vi "Beer_Pong_selecteur.vi"(0 "Espace dispo":dbl[][](array[numeric]), 1 "Timeout Count":u32, 5 "Zone 3":dbl[][](array[numeric]), 7 "Zone 2":dbl[][](array[numeric])=[[0.0, 1.0, 2.0, 3.0, 4.0, 32.0, 33.0, 36.0], [15.0, 30.0, 18.0, 24.0, 26.0, 13.0, 16.0, 19.0], [1.0, 0.0, 0.0, 0.0, 0.0, 0.0, 0.0, 0.0]], 11 "error in (no error)":errorcluster, 12 "Tick Count(mSec)":u32, 13 "New Angle":dbl) -> (4 "Selection de état":T2, 6 "Timeout Count":u32, 8 "Tick Count(mSec)":u32, 10 "New Angle":dbl, 14 "Timeout":bool=TRUE, 15 "error out":errorcluster)   [LabVIEW 2017]
uses:
  enum_etats_lidar.ctl
  enum_etats_beer_pong.ctl
panel:
  in  "Enum etat beer pong":T1
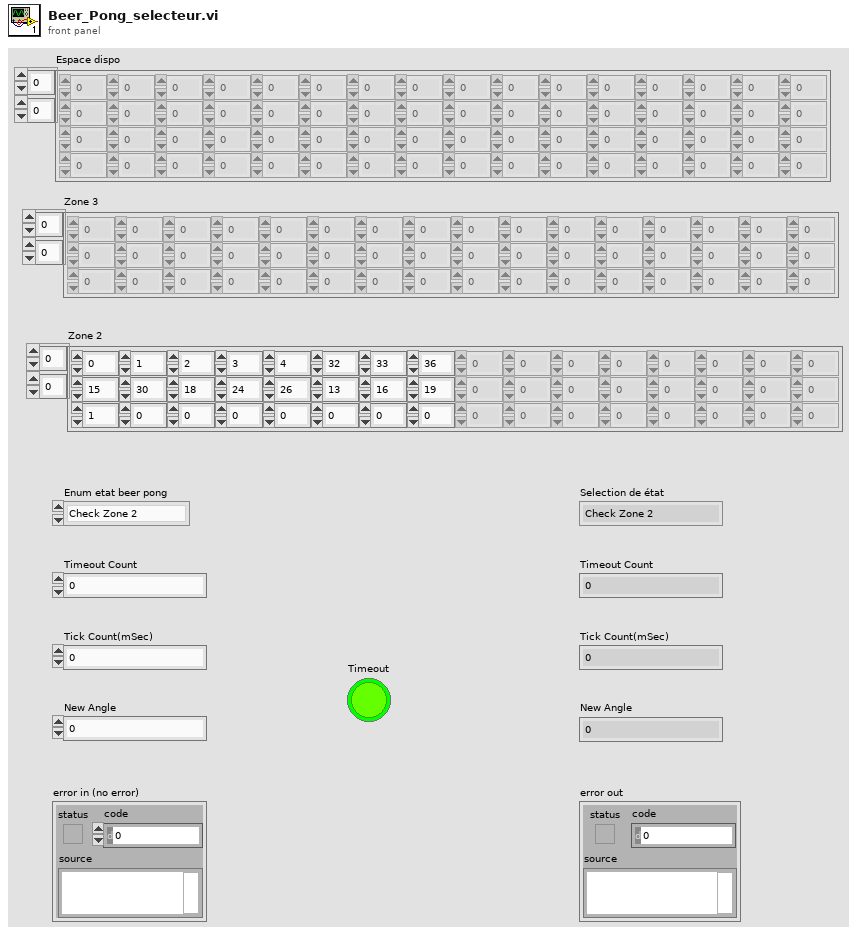
[diagram p1: front panel]
types:
  T1 = typedef "enum_etats_beer_pong.ctl" = enum16{"Check Zone 2", "Obstacle Zone 2", "Check Zone 3", "Obstacle Zone 3", "Avance", "Obstacle Timer", "Rescan 10s", "Check Zone 3 Bis", "Rotation new direction", "Rotation 180", "Timeout ?", "Arret complet", "Rotation new dir timer", "Rotation 180 timer"}
  T2 = typedef "enum_etats_lidar.ctl" = enum16{"Check Zone 2", "Obstacle Zone 2", "Check Zone 3", "Obstacle Zone 3", "Avance", "Obstacle Timer", "Rescan 10s", "Check Zone 3 Bis", "Rotation new direction", "Rotation 180", "Timeout ?", "Arret complet", "Rotation new dir timer", "Rotation 180 timer"}
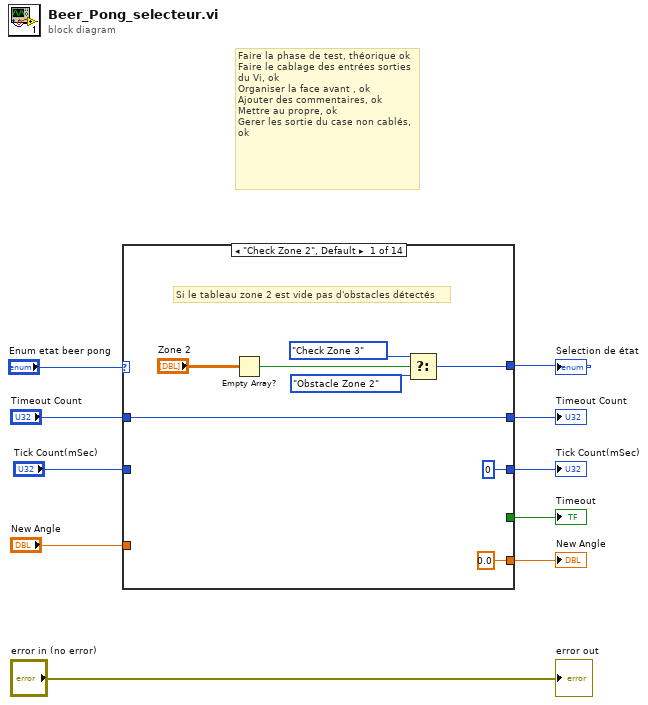
[diagram p0: block diagram]
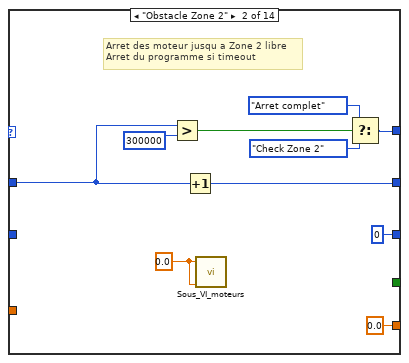
[diagram p2: hidden frame]
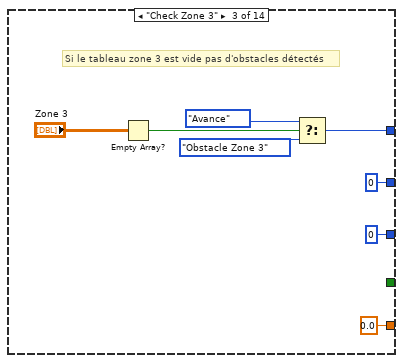
[diagram p3: hidden frame]
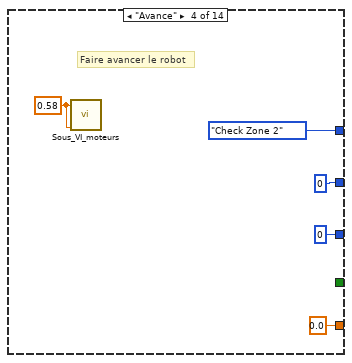
[diagram p4: hidden frame]
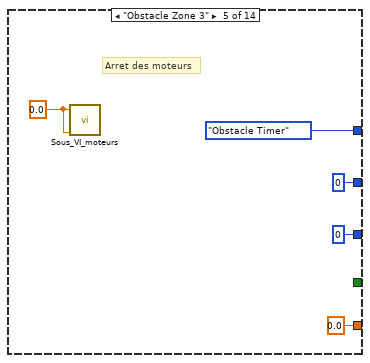
[diagram p5: hidden frame]
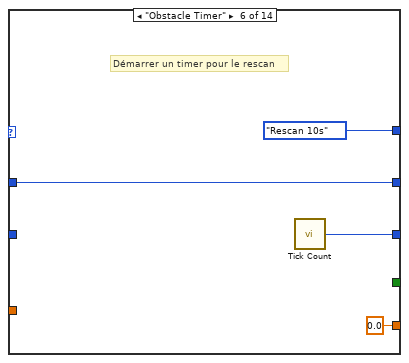
[diagram p6: hidden frame]
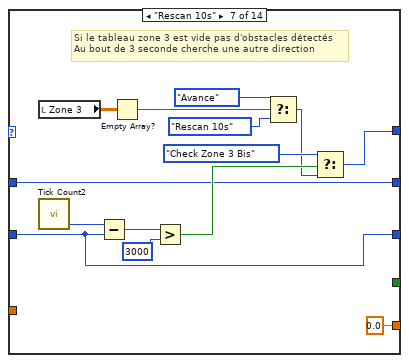
[diagram p7: hidden frame]
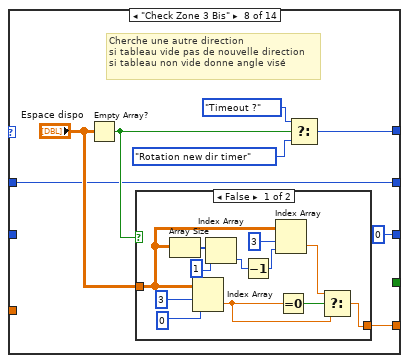
[diagram p8: hidden frame]
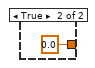
[diagram p9: hidden frame]
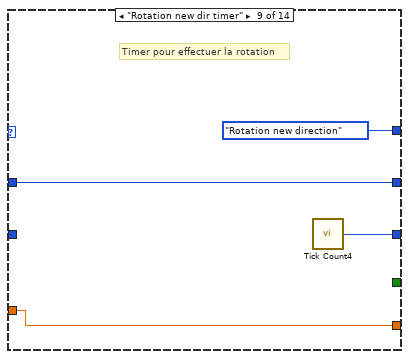
[diagram p10: hidden frame]
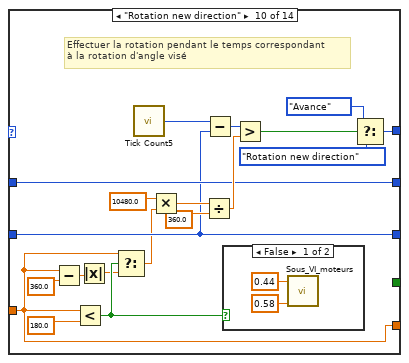
[diagram p11: hidden frame]
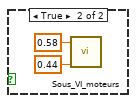
[diagram p12: hidden frame]
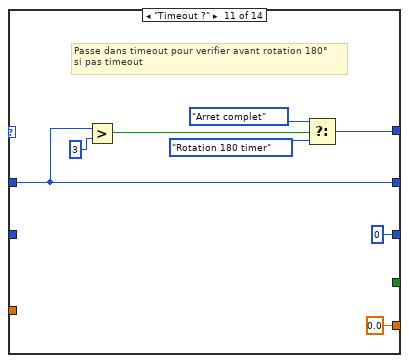
[diagram p13: hidden frame]
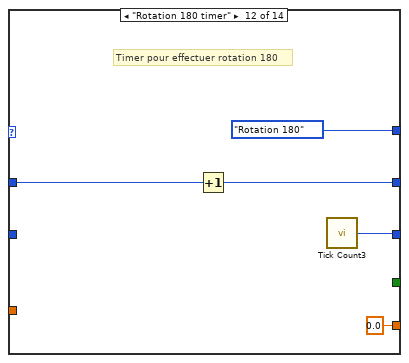
[diagram p14: hidden frame]
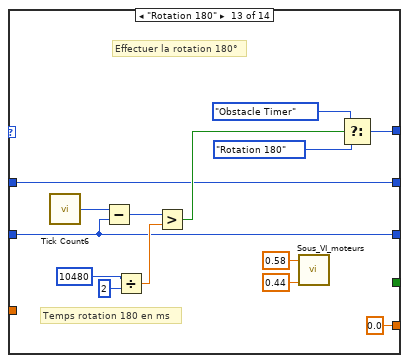
[diagram p15: hidden frame]
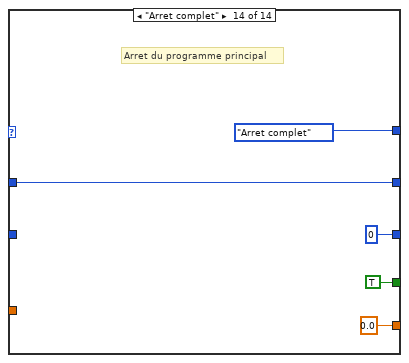
[diagram p16: hidden frame]
diagram:
  # "Faire la phase de test, théorique ok\nFaire le cablage des entrées sorties\ndu Vi, ok\nOrganiser la face avant , ok\nAjouter des commentaires, ok\nMettre au propre, ok\nGerer les sortie du case non cablés, ok"
  n1 = case shown="\"Check Zone 2\", Default" "Enum etat beer pong" {
    tunnel: [w14 w22 w32 enum_etats_lidar."Check Zone 2" ("Enum") enum_etats_lidar."Obstacle Timer" ("Enum") enum_etats_lidar."Rescan 10s" ("Enum") w51 w70 enum_etats_lidar."Rotation new direction" ("Enum") w106 w120 enum_etats_lidar."Rotation 180" ("Enum") w132 enum_etats_lidar."Arret complet" ("Enum")] -> w9
    tunnel: [u32 0 ("Tick Count(mSec)") u32 0 ("Tick Count(mSec)") u32 0 ("Tick Count(mSec)") u32 0 ("Tick Count(mSec)") u32 0 ("Tick Count(mSec)") w50 w53 u32 0 ("Tick Count(mSec)") w88 w98 u32 0 ("Tick Count(mSec) 2") w124 w128 u32 0 ("Tick Count(mSec) 2")] -> w8
    tunnel: "Tick Count(mSec)" -> [_ _ _ _ _ _ w53 _ _ w98 _ _ w128 _]
    tunnel: [_ _ _ _ _ _ _ _ _ _ _ _ _ TRUE] -> w6
    tunnel: "Timeout Count" -> [w11 w23 _ _ _ w48 w54 w66 w87 w99 w115 w121 w126 w142]
    tunnel: [w11 w24 0 0 ("Timeout Count") 0 w48 w54 w66 w87 w99 w115 w122 w126 w142] -> w4
    tunnel: [0.0 ("New Angle") 0.0 ("New Angle") 0.0 ("New Angle") 0.0 ("New Angle") 0.0 ("New Angle") 0.0 ("New Angle") 0.0 ("New Angle") w68 w86 w91 0.0 ("New Angle") 0.0 ("New Angle") 0.0 ("New Angle") 0.0 ("New Angle")] -> w3
    tunnel: "New Angle" -> [_ _ _ _ _ _ _ _ w86 w91 _ _ _ _]
    frame "Check Zone 2", Default {
      # "Si le tableau zone 2 est vide pas d'obstacles détectés"
      n2 = Empty Array?(array="Zone 2") -> (empty?=w17:bool)
      n3 = Select(t=enum_etats_lidar."Check Zone 3" ("Enum"), s=w17, f=enum_etats_lidar."Obstacle Zone 2" ("Enum")) -> (s? t:f=w14:T2)
    }
    frame "Obstacle Zone 2" {
      w28 = 0.0 ("Moteur Gauche")
      # "Arret des moteur jusqu a Zone 2 libre\nArret du programme si timeout"
      n4 = Greater?(x=w23, y=u32 300000) -> (0:w19:bool)
      n5 = Increment(x=w23) -> (x+1=w24:u32)
      n6 = call "Sous_VI_moteurs.vi"("Moteur Droit"=w28, "Moteur Gauche"=w28) -> ()  [unwired: 10 in]
      n7 = Select(t=enum_etats_lidar."Arret complet" ("Enum"), s=w19, f=enum_etats_lidar."Check Zone 2" ("Enum")) -> (s? t:f=w22:T2)
    }
    frame "Check Zone 3" {
      # "Si le tableau zone 3 est vide pas d'obstacles détectés"
      n8 = Empty Array?(array="Zone 3") -> (empty?=w36:bool)
      n9 = Select(t=enum_etats_lidar."Avance" ("Enum"), s=w36, f=enum_etats_lidar."Obstacle Zone 3" ("Enum")) -> (s? t:f=w32:T2)
    }
    frame "Avance" {
      w40 = 0.58 ("Moteur Gauche")
      # "Faire avancer le robot"
      n10 = call "Sous_VI_moteurs.vi"("Moteur Droit"=w40, "Moteur Gauche"=w40) -> ()  [unwired: 10 in]
    }
    frame "Obstacle Zone 3" {
      w46 = 0.0 ("Moteur Gauche")
      # "Arret des moteurs"
      n11 = call "Sous_VI_moteurs.vi"("Moteur Droit"=w46, "Moteur Gauche"=w46) -> ()  [unwired: 10 in]
    }
    frame "Obstacle Timer" {
      # "Démarrer un timer pour le rescan"
      n12 = call "Tick Count"() -> ("Tick Count(mSec)"=w50:u32)
    }
    frame "Rescan 10s" {
      # "Si le tableau zone 3 est vide pas d'obstacles détectés\nAu bout de 3 seconde cherche une autre direction"
      n13 = local read "Zone 3"() -> (w61:dbl[][])
      n14 = call "Tick Count2"() -> ("Tick Count(mSec)"=w60:u32)
      n15 = Subtract(x=w60, y=w53) -> (x-y=w59:u32)
      n16 = Empty Array?(array=w61) -> (empty?=w64:bool)
      n17 = Greater?(x=w59, y=u32 3000) -> (0:w57:bool)
      n18 = Select(t=enum_etats_lidar."Avance" ("Enum"), s=w64, f=enum_etats_lidar."Rescan 10s" ("Enum")) -> (s? t:f=w55:T2)
      n19 = Select(t=enum_etats_lidar."Check Zone 3 Bis" ("Enum"), s=w57, f=w55) -> (s? t:f=w51:T2)
    }
    frame "Check Zone 3 Bis" {
      # "Cherche une autre direction\nsi tableau vide pas de nouvelle direction\nsi tableau non vide donne angle visé"
      n20 = Empty Array?(array="Espace dispo") -> (empty?=w69:bool)
      n21 = case shown="False" w69 {
        tunnel: [w78 0.0 ("Numeric")] -> w68
        tunnel: "Espace dispo" -> [w77 _]
        frame False {
          n22 = Array Size(array=w77) -> (size(s)=w76:i32[])
          n23 = Index Array(array=w77, index (row)=3, index (col)=0 ("disabled index (col)")) -> (element=w81:dbl)
          n24 = Index Array(array=w76, index=1) -> (element=w73:i32)
          n25 = Decrement(x=w73) -> (x-1=w74:i32)
          n26 = Index Array(array=w77, index (row)=3, index (col)=w74) -> (element=w79:dbl)
          n27 = Equal To 0?(x=w81) -> (x = 0?=w82:bool)
          n28 = Select(t=w79, s=w82, f=w81) -> (s? t:f=w78:dbl)
        }
        frame True {
        }
      }
      n29 = Select(t=enum_etats_lidar."Timeout ?" ("Enum"), s=w69, f=enum_etats_lidar."Rotation new dir timer" ("Enum")) -> (s? t:f=w70:T2)
    }
    frame "Rotation new dir timer" {
      # "Timer pour effectuer la rotation"
      n30 = call "Tick Count4"() -> ("Tick Count(mSec)"=w88:u32)
    }
    frame "Rotation new direction" {
      # "Effectuer la rotation pendant le temps correspondant \nà la rotation d'angle visé"
      n31 = Subtract(x=w91, y=360.0) -> (x-y=w92:dbl)
      n32 = Less?(x=w91, y=180.0) -> (x < y?=w96:bool)
      n33 = Absolute Value(x=w92) -> (abs(x)=w93:dbl)
      n34 = Select(t=w91, s=w96, f=w93) -> (s? t:f=w94:dbl)
      n35 = call "Tick Count5"() -> ("Tick Count(mSec)"=w97:u32)
      n36 = Multiply(x=10480.0, y=w94) -> (x*y=w102:dbl)
      n37 = Divide(x=w102, y=360.0) -> (x/y=w101:dbl)
      n38 = Subtract(x=w97, y=w98) -> (x-y=w108:u32)
      n39 = case shown="False" w96 {
        frame False {
          n40 = call "Sous_VI_moteurs.vi"("Moteur Droit"=0.58, "Moteur Gauche"=0.44) -> ()  [unwired: 10 in]
        }
        frame True {
          n41 = call "Sous_VI_moteurs.vi"("Moteur Droit"=0.44, "Moteur Gauche"=0.58) -> ()  [unwired: 10 in]
        }
      }
      n42 = Greater?(x=w108, y=w101) -> (0:w107:bool)
      n43 = Select(t=enum_etats_lidar."Avance" ("Enum"), s=w107, f=enum_etats_lidar."Rotation new direction" ("Enum")) -> (s? t:f=w106:T2)
    }
    frame "Timeout ?" {
      # "Passe dans timeout pour verifier avant rotation 180°\nsi pas timeout"
      n44 = Greater?(x=w115, y=3) -> (0:w117:bool)
      n45 = Select(t=enum_etats_lidar."Arret complet" ("Enum"), s=w117, f=enum_etats_lidar."Rotation 180 timer" ("Enum")) -> (s? t:f=w120:T2)
    }
    frame "Rotation 180 timer" {
      # "Timer pour effectuer rotation 180"
      n46 = Increment(x=w121) -> (x+1=w122:u32)
      n47 = call "Tick Count3"() -> ("Tick Count(mSec)"=w124:u32)
    }
    frame "Rotation 180" {
      # "Temps rotation 180 en ms"
      # "Effectuer la rotation 180°"
      n48 = call "Tick Count6"() -> ("Tick Count(mSec)"=w137:u32)
      n49 = Subtract(x=w137, y=w128) -> (x-y=w136:u32)
      n50 = Divide(x=u32 10480 ("y"), y=u32 2) -> (x/y=w129:dbl)
      n51 = Greater?(x=w136, y=w129) -> (0:w135:bool)
      n52 = call "Sous_VI_moteurs.vi"("Moteur Droit"=0.44, "Moteur Gauche"=0.58) -> ()  [unwired: 10 in]
      n53 = Select(t=enum_etats_lidar."Obstacle Timer" ("Enum"), s=w135, f=enum_etats_lidar."Rotation 180" ("Enum")) -> (s? t:f=w132:T2)
    }
    frame "Arret complet" {
      # "Arret du programme principal"
    }
  }
  "Selection de état" <- w9
  "Tick Count(mSec)" <- w8
  "Timeout" <- w6
  "Timeout Count" <- w4
  "New Angle" <- w3
  "error out" <- "error in (no error)"
